vi "Compare Variant Types.vi"(8 "error in (no error)":errorcluster, 10 "Variant 2":variant, 11 "Variant":variant) -> (0 "error out":errorcluster, 3 "Variants have compatible types ?":bool)   [LabVIEW 2012, in "Scripting Tools.lvlib"]
uses:
  <userlib>/_LAVAcr/Scripting Tools/Scripting Tools.lvlib
  <vilib>/Utility/VariantDataType/VariantType.lvlib
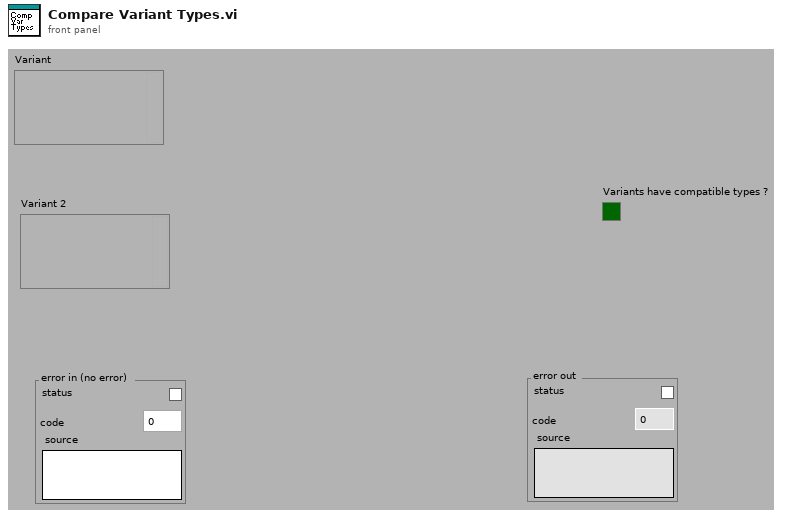
[diagram p1: front panel]
types:
  T1 = typedef "VariantType.lvlib/Type.ctl" = enum8{"Invalid Type", "Void", "I8", "I16", "I32", "I64", "U8", "U16", "U32", "U64", "Single Float", "Double Float", "Extended Float", "Single Complex", "Double Complex", "Extended Complex", "Enum U8", "Enum U16", "Enum U32", "Enum U64", "Single Float With Unit", "Double Float With Unit", "Extended Float With Unit", "Single Complex with Unit", "Double Complex with Unit", "Extended Complex with Unit", "Boolean", "String", "Path", "Picture", "Tag", "Array", "Cluster", "Variant", "LV Variant", "Waveform", "Timestamp", "Digital Waveform", "Digital Data", "ExpressData", "Refnum", "External Data", "VI", "Poly VI", "LabVIEW Class Instance", "Fixed Point"}
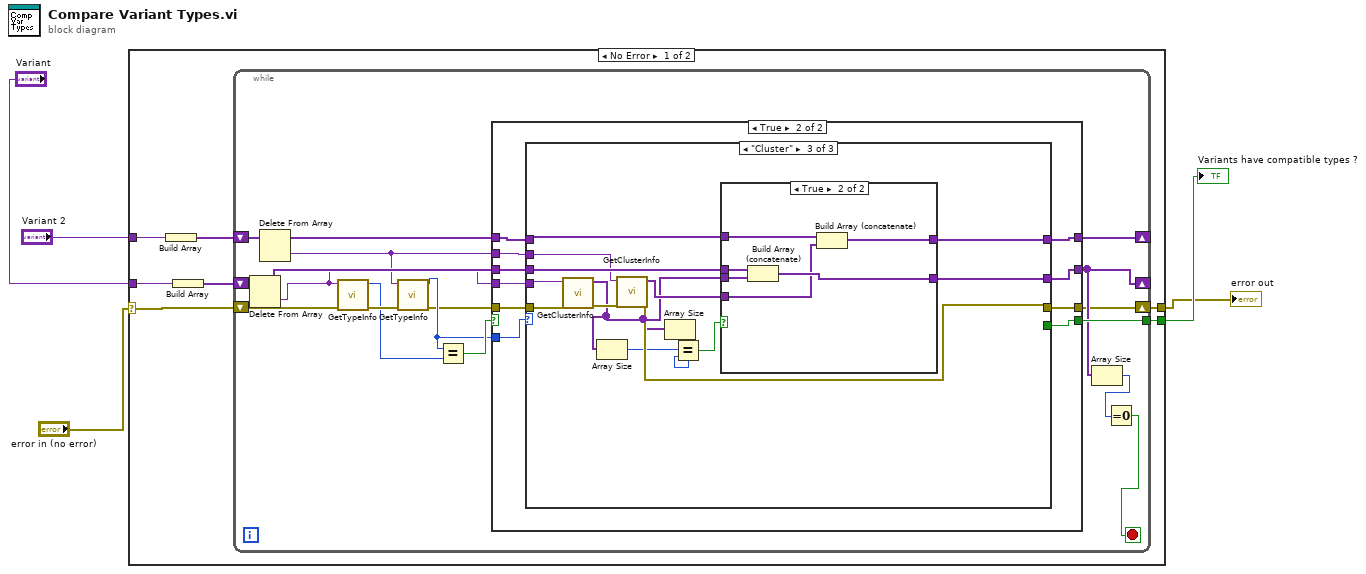
[diagram p0: block diagram]
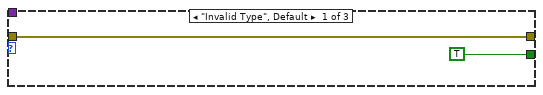
[diagram p3: hidden frame]
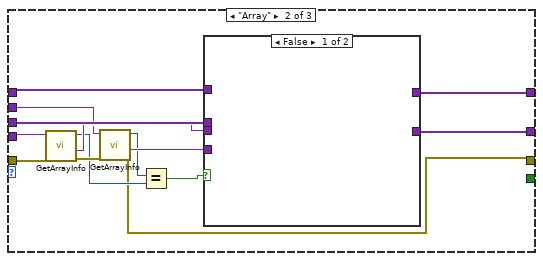
[diagram p4: hidden frame]
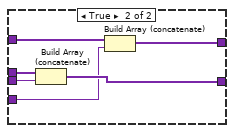
[diagram p5: hidden frame]
diagram:
  n1 = case shown="No Error" "error in (no error)" {
    selector: "error in (no error)" -> [w12 w85]
    tunnel: "Variant" -> [w11 _]
    tunnel: "Variant 2" -> [w10 _]
    tunnel: [w9 _] -> w2
    tunnel: [w6 w85] -> w1
    frame No Error {
      n2 = Build Array(w10) -> (w8:variant[])
      n3 = Build Array(w11) -> (w7:variant[])
      n4 = while {
        tunnel: [w24] -> w9
        shift-right: [w22] -> _
        shift-left: w8 -> [w27]
        shift-right: [w19] -> _
        shift-left: w7 -> [w29]
        shift-right: [w16] -> w6
        shift-left: w12 -> [w30]
        stop <- w17 stop-if-true
        n5 = Delete From Array(array=w29) -> (deleted portion=w13:variant, array with subset deleted=w21:variant[])  [unwired: 2 in]
        n6 = Delete From Array(array=w27) -> (deleted portion=w14:variant, array with subset deleted=w23:variant[])  [unwired: 2 in]
        n7 = call <vilib>:"GetTypeInfo.vi"("error in (no error)"=w30, "Variant"=w13) -> ("error out"=w28:errorcluster, "Type Enum"=w26:T1)  [unwired: 8 out]
        n8 = call <vilib>:"GetTypeInfo.vi"("error in (no error)"=w28, "Variant"=w14) -> ("error out"=w15:errorcluster, "Type Enum"=w20:T1)  [unwired: 8 out]
        n9 = Equal?(x=w20, y=w26) -> (x = y?=w25:bool)
        n10 = case shown="True" w25 {
          selector: w25 -> [w32 _]
          tunnel: [w32 w37] -> w24
          tunnel: w23 -> [_ w41]
          tunnel: [_ w40] -> w22
          tunnel: [_ w39] -> w19
          tunnel: w21 -> [_ w38]
          tunnel: w20 -> [_ w42]
          tunnel: [w31 w36] -> w16
          tunnel: w15 -> [w31 w35]
          tunnel: w14 -> [_ w34]
          tunnel: w13 -> [_ w33]
          frame False {
          }
          frame True {
            n11 = case shown="\"Cluster\"" w42 {
              tunnel: w41 -> [_ w51 w72]
              tunnel: [_ w49 w71] -> w40
              tunnel: [_ w55 w75] -> w39
              tunnel: w38 -> [_ w58 w78]
              tunnel: [TRUE _ _] -> w37
              tunnel: [w43 w45 w69] -> w36
              tunnel: w35 -> [w43 w57 w77]
              tunnel: w34 -> [_ w52 w73]
              tunnel: w33 -> [_ w56 w76]
              frame "Invalid Type", Default {
              }
              frame "Array" {
                n12 = call <vilib>:"GetArrayInfo.vi"("error in (no error)"=w57, "Variant"=w56) -> ("error out"=w54:errorcluster, "ArrayElement"=w53:variant, "NDims"=w47:i32)  [unwired: 7 out]
                n13 = call <vilib>:"GetArrayInfo.vi"("error in (no error)"=w54, "Variant"=w52) -> ("error out"=w45:errorcluster, "ArrayElement"=w50:variant, "NDims"=w48:i32)  [unwired: 7 out]
                n14 = Equal?(x=w48, y=w47) -> (x = y?=w46:bool)
                n15 = case shown="False" w46 {
                  tunnel: w58 -> [_ w64]
                  tunnel: [_ w63] -> w55
                  tunnel: w53 -> [_ w62]
                  tunnel: w51 -> [_ w61]
                  tunnel: w50 -> [_ w60]
                  tunnel: [_ w59] -> w49
                  frame False {
                  }
                  frame True {
                    n16 = Build Array (concatenate)(w64, w62) -> (w63:variant[])
                    n17 = Build Array (concatenate)(w61, w60) -> (w59:variant[])
                  }
                }
              }
              frame "Cluster" {
                n18 = call <vilib>:"GetClusterInfo.vi"("error in (no error)"=w77, "Variant"=w76) -> ("error out"=w74:errorcluster, "Cluster Elements"=w66:variant[])  [unwired: 8 out]
                n19 = Array Size(array=w66) -> (size(s)=w67:i32)
                n20 = call <vilib>:"GetClusterInfo.vi"("error in (no error)"=w74, "Variant"=w73) -> ("error out"=w69:errorcluster, "Cluster Elements"=w68:variant[])  [unwired: 8 out]
                n21 = Array Size(array=w66) -> (size(s)=w65:i32)
                n22 = Equal?(x=w67, y=w65) -> (x = y?=w70:bool)
                n23 = case shown="True" w70 {
                  tunnel: w78 -> [_ w84]
                  tunnel: [_ w83] -> w75
                  tunnel: w66 -> [_ w82]
                  tunnel: w72 -> [_ w81]
                  tunnel: w68 -> [_ w80]
                  tunnel: [_ w79] -> w71
                  frame False {
                  }
                  frame True {
                    n24 = Build Array (concatenate)(w84, w82) -> (w83:variant[])
                    n25 = Build Array (concatenate)(w81, w80) -> (w79:variant[])
                  }
                }
              }
            }
          }
        }
        n26 = Array Size(array=w19) -> (size(s)=w18:i32)
        n27 = Equal To 0?(x=w18) -> (x = 0?=w17:bool)
      }
    }
    frame Error {
    }
  }
  "error out" <- w1
  "Variants have compatible types ?" <- w2
